vi "fake prompt required argument.vi"(10 "style":string, 11 "topic":string) -> (3 "prompt":string)   [LabVIEW 2020, in "MCP Server tests.lvlib"]
doc: "This is a fake prompt to test the MCP server toolkit. It has one required argument (topic) and one optional argument (style)."
uses:
  MCP Server tests.lvlib
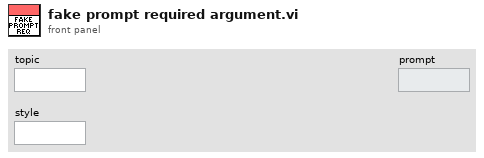
[diagram p1: front panel]
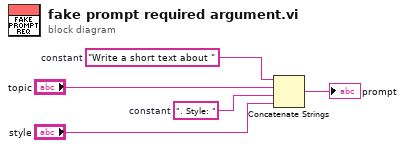
[diagram p0: block diagram]
diagram:
  w3 = ". Style: "  # constant
  w5 = "Write a short text about "  # constant
  n1 = Concatenate Strings(w5, "topic", w3, "style") -> (→"prompt":string)
